vi "TCP Write Bytes.vi"(8 "error in (no error)":errorcluster, 9 "timeout ms (2000)":i32=2000, 10 "Bytes":u8[](array[numeric]) format="%08b", 11 "Connection.TCP":refnum<class "Connection.TCP.lvclass">) -> (0 "error out":errorcluster, 3 "Connection.TCP":refnum<class "Connection.TCP.lvclass">)   [LabVIEW 2013, in "Connection.TCP_GOSPL.lvlib" / "Connection.TCP.lvclass"]
uses:
  Connection.TCP.lvclass
  Connection.TCP.lvclass/Connection.TCP.ctl
  Connection/Connection.lvclass
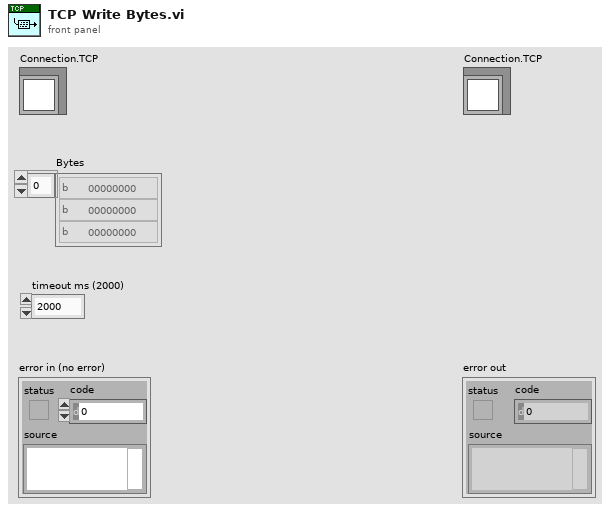
[diagram p1: front panel]
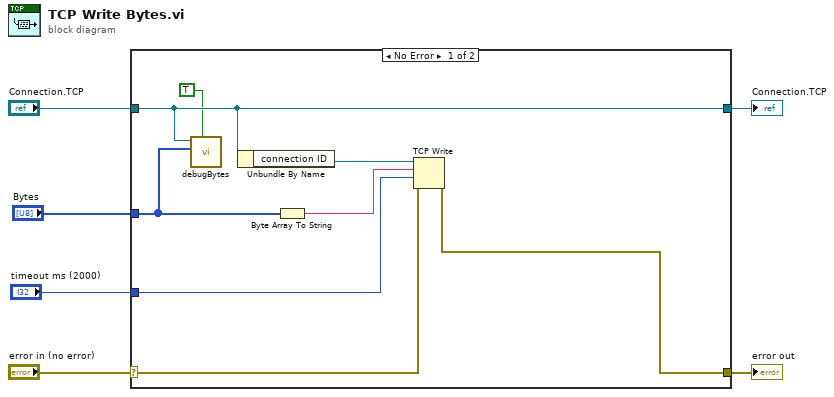
[diagram p0: block diagram]
diagram:
  n1 = case shown="No Error" "error in (no error)" {
    selector: "error in (no error)" -> [w12 w16]
    tunnel: [w11 w16] -> w5
    tunnel: [w9 w15] -> w3
    tunnel: "Connection.TCP" -> [w9 w15]
    tunnel: "Bytes" -> [w8 _]
    tunnel: "timeout ms (2000)" -> [w10 _]
    frame No Error {
      n2 = call "debugBytes.vi"("outgoing?"=TRUE, "Bytes"=w8, "Connection in"=w9) -> ()  [unwired: 7 in, 2 out]
      n3 = Unbundle By Name(w9) -> ("connection ID"=w14:refnum<k5>)
      n4 = Byte Array To String(unsigned byte array=w8) -> (string=w13:string)
      n5 = TCP Write(connection ID=w14, data in=w13, error in (no error)=w12, 9:w10) -> (error out=w11:errorcluster)  [unwired: 2 out]
    }
    frame Error {
    }
  }
  "error out" <- w5
  "Connection.TCP" <- w3
